vi "xnet_canopen_set_fault.vi"(6 "active":u8, 7 "info_code":u32, 8 "error in (no error)":errorcluster, 9 "error_code":u16, 10 "error_bit":u8, 11 "xnet_co_handle_in":u64) -> (0 "error out":errorcluster, 3 "xnet_co_handle":u64)   [LabVIEW 2023, in "xnet_canopen.lvlib"]
uses:
  <vilib>/Utility/error.llb/Error Cluster From Error Code.vi
  xnet_canopen.lvlib
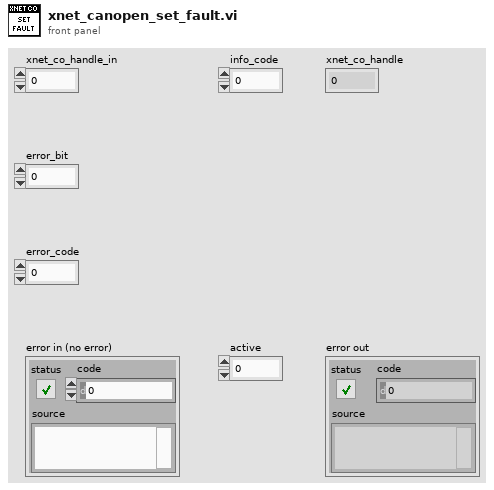
[diagram p1: front panel]
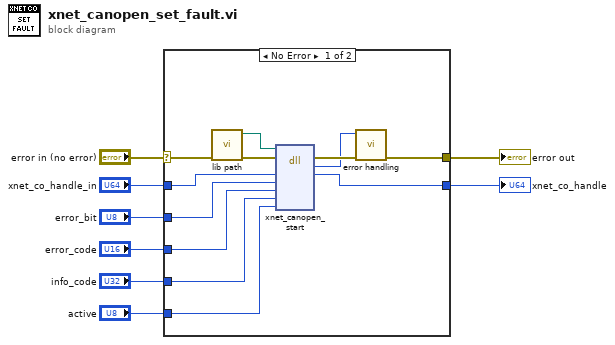
[diagram p0: block diagram]
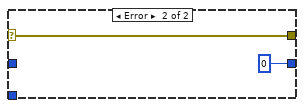
[diagram p2: hidden frame]
diagram:
  n1 = case shown="No Error" "error in (no error)" {
    selector: "error in (no error)" -> [w18 w21]
    tunnel: [w16 w21] -> w7
    tunnel: [w14 u64 0 ("phandle")] -> w6
    tunnel: "xnet_co_handle_in" -> [w13 _]
    tunnel: "error_bit" -> [w12 _]
    tunnel: "error_code" -> [w11 _]
    tunnel: "info_code" -> [w10 _]
    tunnel: "active" -> [w9 _]
    frame No Error {
      n2 = call "lib path.vi"() -> ("lib path"=w19:path)  [unwired: 11 in]
      n3 = dll-call lib="?" fn="xnet_canopen_start"(path in=w19, error in=w18, "handle"=w13, "error_bit"=w12, "error_code"=w11, "info_code"=w10, "active"=w9) -> (error out=w17:errorcluster, "return type"=w15:i32, "handle"=w14:u64)  [unwired: 5 in, 1 out]
      n4 = call "error handling.vi"("error in (no error)"=w17, "return val"=w15) -> ("error out"=w16:errorcluster)  [unwired: 9 in]
    }
    frame Error {
    }
  }
  "error out" <- w7
  "xnet_co_handle" <- w6
